vi "Measure.vi"(8 "error in (no error)":errorcluster, 11 "Prototype Measurement in":refnum<class "Prototype Measurement.lvclass">) -> (0 "error out":errorcluster, 3 "Prototype Measurement out":refnum<class "Prototype Measurement.lvclass">)   [LabVIEW 2016]
uses:
  user.lib/Common Components/Results/Results.lvclass
  Result/Prototype Result.lvclass
  C:/Program Files (x86)/National Instruments/LabVIEW 2016/user.lib/Common Components/Results/Results.lvclass
  user.lib/Common Components/Measurement Actor/Measurement.lvclass
  Measurement/Prototype Measurement.lvclass
  C:/Program Files (x86)/National Instruments/LabVIEW 2016/user.lib/Common Components/Measurement Actor/Measurement.lvclass
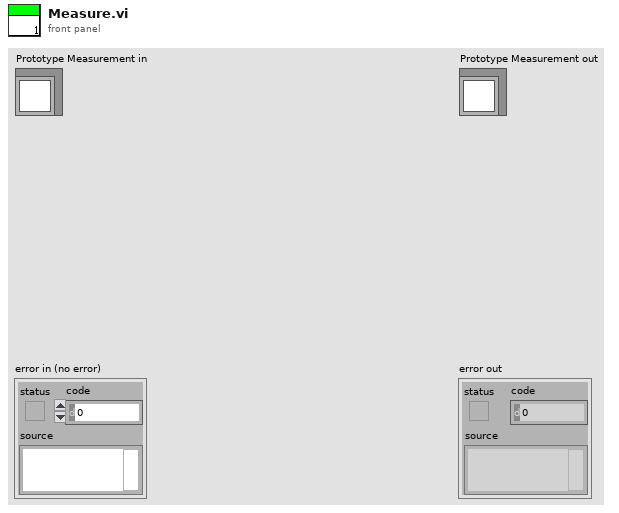
[diagram p1: front panel]
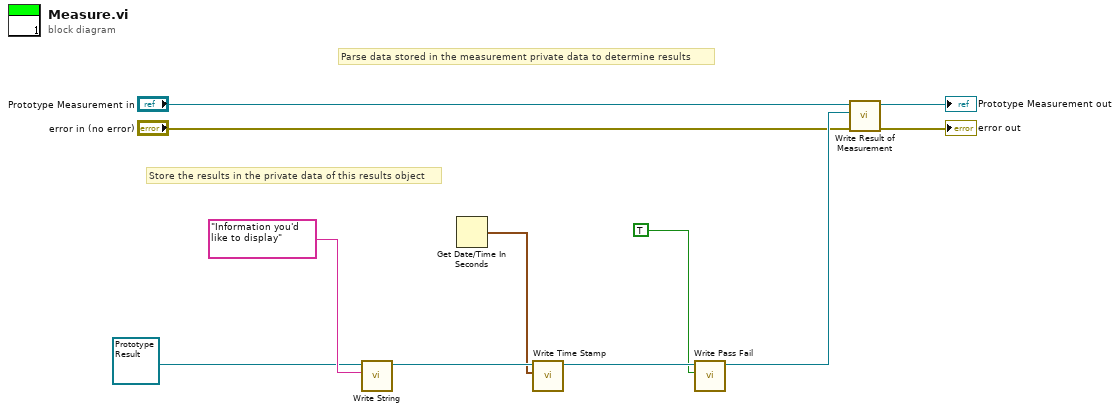
[diagram p0: block diagram]
diagram:
  # "Store the results in the private data of this results object"
  # "Parse data stored in the measurement private data to determine results"
  n1 = call "Write String.vi"("String"="Information you'd like to display", "Results in"=refnum<class "Prototype Result.lvclass"> refnum ("Prototype Result.lvclass")) -> ("Results out"=w11:refnum<class "Prototype Result.lvclass">)  [unwired: 8 in, 1 out]
  n2 = Get Date/Time In Seconds() -> (seconds since 1Jan1904=w8:timestamp)
  n3 = call "Write Time Stamp.vi"("Time Stamp"=w8, "Results in"=w11) -> ("Results out"=w10:refnum<class "Prototype Result.lvclass">)  [unwired: 8 in, 1 out]
  n4 = call "Write Pass Fail.vi"("Pass Fail"=TRUE, "Results in"=w10) -> ("Results out"=w5:refnum<class "Prototype Result.lvclass">)  [unwired: 8 in, 1 out]
  n5 = call "Write Result of Measurement.vi"("error in (no error)"="error in (no error)", "Result Actor.lvlib:Results.lvclass"=w5, "Measurement in"="Prototype Measurement in") -> ("error out"=→"error out":errorcluster, "Measurement out"=→"Prototype Measurement out":refnum<class "Prototype Measurement.lvclass">)  [unwired: 7 in]
